vi "Read Bus Monitor ID.vi"(11 "IBusMonitor":refnum<class "IBusMonitor.lvclass">) -> (3 "Bus Monitor ID":string)   [LabVIEW 2018, in "MVA Framework.lvlib" / "MonitoredMediator.lvlib" / "IBusMonitor.lvclass"]
uses:
  IBusMonitor.lvclass
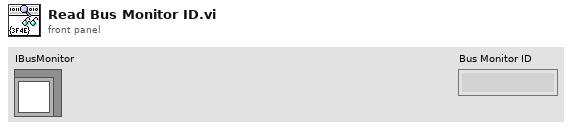
[diagram p1: front panel]
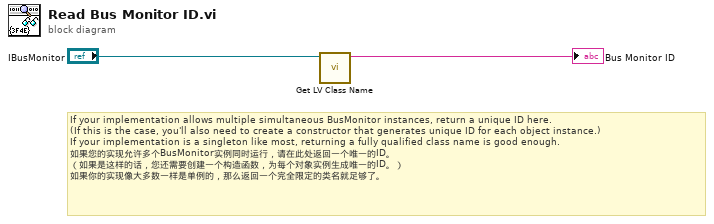
[diagram p0: block diagram]
diagram:
  # "If your implementation allows multiple simultaneous BusMonitor instances, return a unique ID here.\n(If this is the case, you'll also need to create a constructor that generates unique ID for each object instance.)\nIf your implementation is a singleton like most, returning a fully qualified class name is good enough.\n如果您的实现允许多个BusMonitor实例同时运行，请在此处返回一个唯一的ID。\n（如果是这样的话，您还需要创建一个构造函数，为每个对象实例生成唯一的ID。）\n如果你的实现像大多数一样是单例的，那么返回一个完全限定的类名就足够了。"
  n1 = call <vilib>:"Get LV Class Name.vi"("object"="IBusMonitor") -> ("class name"=→"Bus Monitor ID":string)  [unwired: 9 in, 1 out]
